vi "Constructor.vi"(6 "Database_path":path=path "D:/Sgraph_database", 8 "error in (no error)":errorcluster, 9 "DAQ-Queue":refnum<queue>, 10 "Gserver-Queue":refnum<queue>, 11 "FAMM in":refnum<class "FAMM.lvclass">) -> (0 "error out":errorcluster, 3 "FAMM out":refnum<class "FAMM.lvclass">, 5 "Layers":i32, 7 "Resolution":dbl format="%.3f")   [LabVIEW 2020, in "Sgraph_lib_V1.lvlib" / "FAMM.lvclass"]
doc: "The FAMM constructor has to be run once in order to set all historian configurations from ini files and to make all memory layer instances. Also the DBAL database type instance is created here. The FAMM object contains all references to FAMM memory and DBAL database methods."
uses:
  FAMM.lvclass
  Gserver/controls/Typedef_Gviewer-Query.ctl
  Gserver/controls/Typedef_QueryType.ctl
  HISW/controls/typedef-DAQ-datagram.ctl
  HISW/controls/typedef-Qtype.ctl
  controls/FAMM-attributes.ctl
  Common/controls/typedef_com_TagProp.ctl
  DBAL/DBAL.lvclass
  PAQ-memory.lvclass
  DBAL/controls/DBAL_Command.ctl
  DBAL/controls/DBAL-commands.ctl
  FAMM.lvclass/FAMM.ctl
  Common/controls/Global-services.vi
  Builds/Sgraph_lib_V1.lvlib
  Gserver/Gserver.lvclass
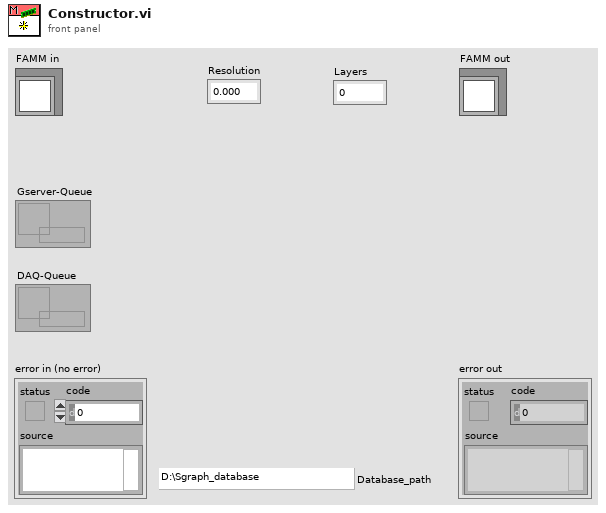
[diagram p1: front panel]
types:
  T1 = typedef "Sgraph_lib_V1.lvlib/FAMM.lvclass/FAMM-attributes.ctl" = cluster{"FAMM_PAQ_Layers":i32, "FAMM_PAQ_resolution":dbl, "PAQ_TAGs":string[], "WAQ_TAGs":string[], "EAQ_TAGs":string[], "All_TAGs":string[], "PAQtagProps":T2[], "WAQtagProps":T2[], "EAQtagProps":T2[], "DBAL_class":refnum<data-value>, "PAQ_memory":refnum<data-value>[], "PAQupdates":timestamp[], "FAMM_Size":cluster{"other":i32, "1day":i32, "1week":i32}, "DatabaseFileExtention":string, "DatabaseSaveRate":dbl, "Database_path":path, "DBAL-Queue":refnum<queue>}
  T2 = typedef "Sgraph_lib_V1.lvlib/typedef_com_TagProp.ctl" = cluster{"Description":string, "EngUnits":string, "RangeH":dbl, "RangeL":dbl, "Resolution":i32, "Obsolete":bool, "ChangeDate":timestamp, "ChangeSource":string, "ChangeReason":string, "TagFunc":u32}
  T3 = cluster{"Size":i32, "Layer":i32, "TableName":string, "LayersQTY":i32, "Skip":i32}
  T4 = typedef "Sgraph_lib_V1.lvlib/DBAL_TAGprops.ctl" = T5[]
  T5 = typedef "Sgraph_lib_V1.lvlib/DBAL_TAGpropEdit.ctl" = cluster{"TAG":string, "Qtype":string, "TAGprop":T2}
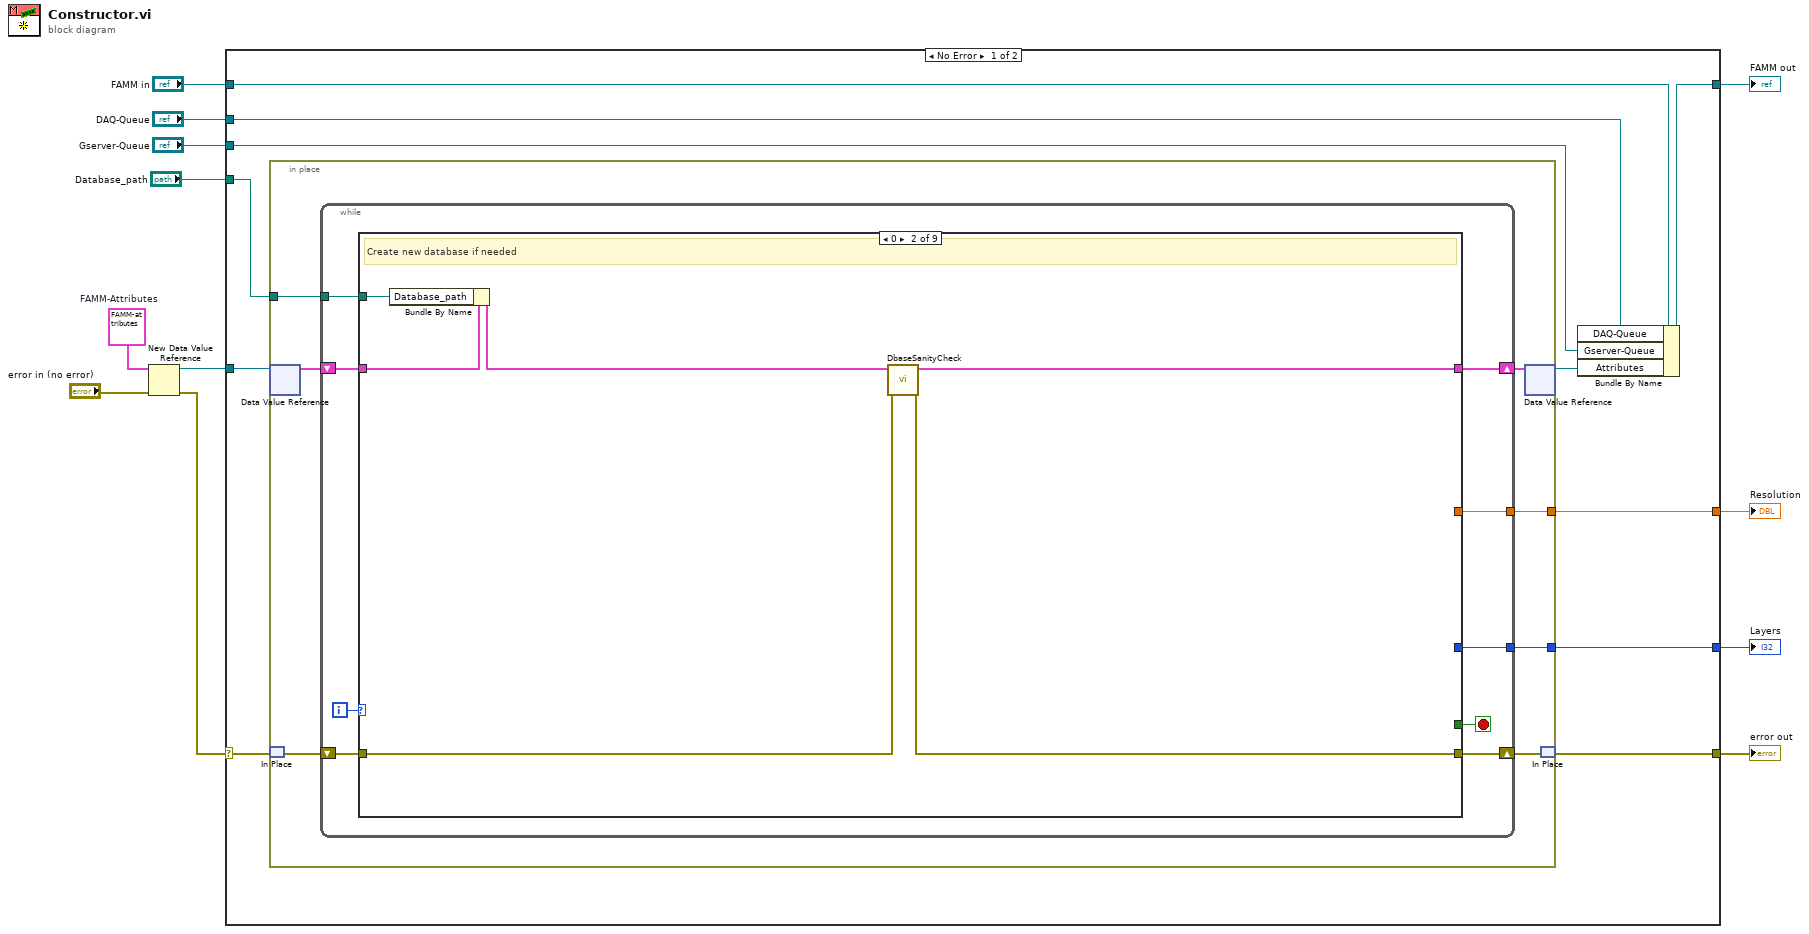
[diagram p0: block diagram]
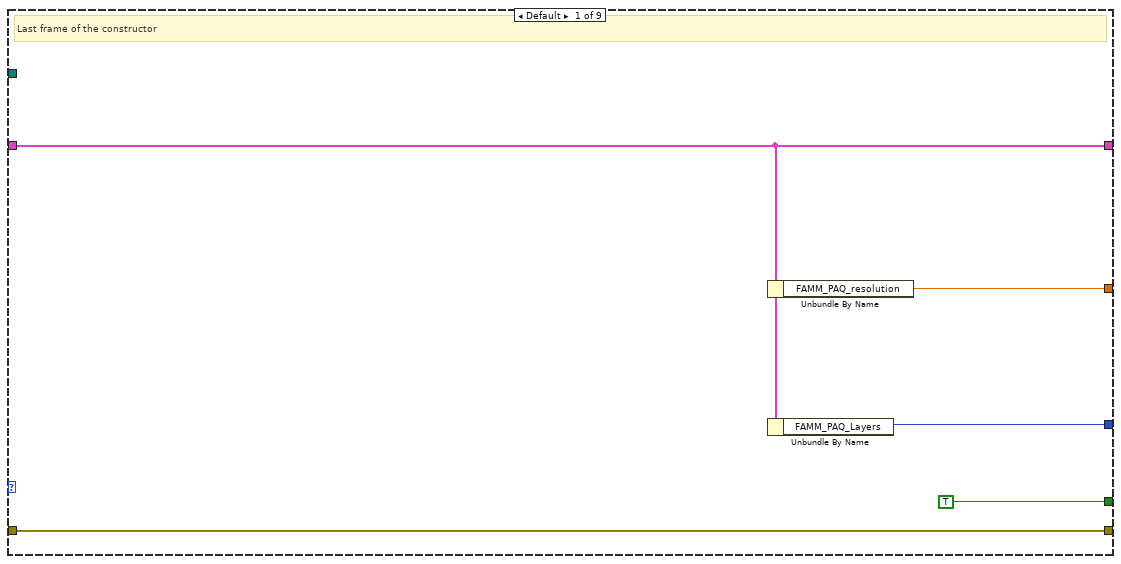
[diagram p2: hidden frame]
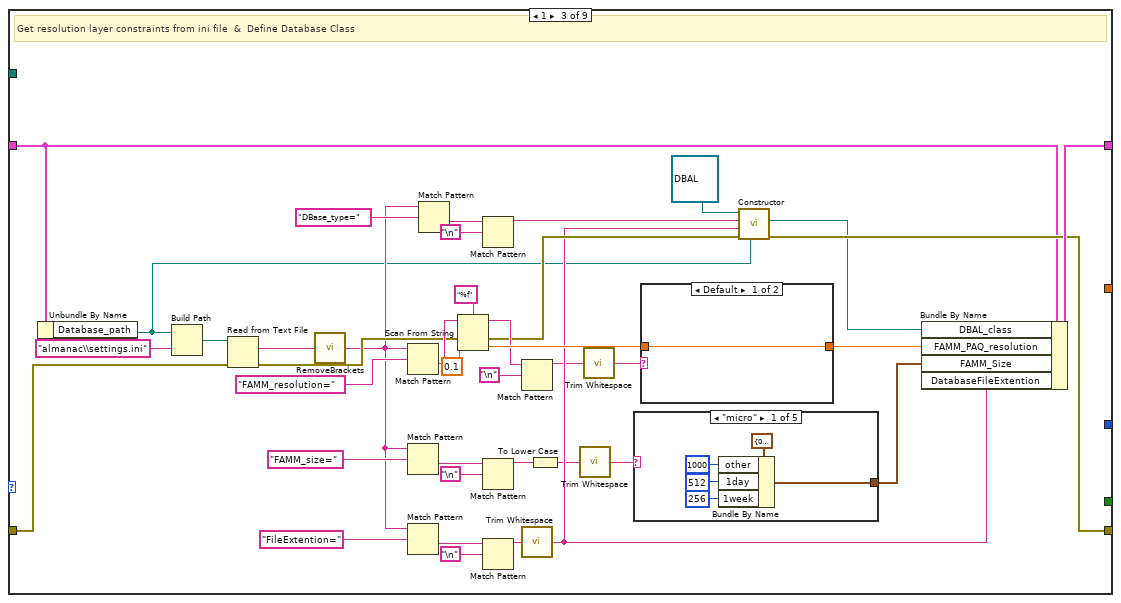
[diagram p3: hidden frame]
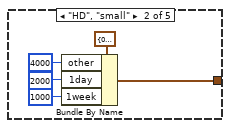
[diagram p4: hidden frame]
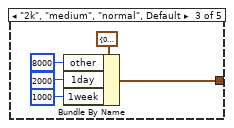
[diagram p5: hidden frame]
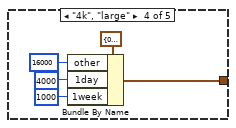
[diagram p6: hidden frame]
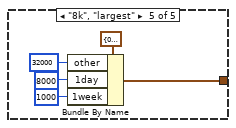
[diagram p7: hidden frame]
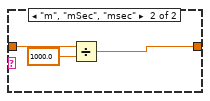
[diagram p8: hidden frame]
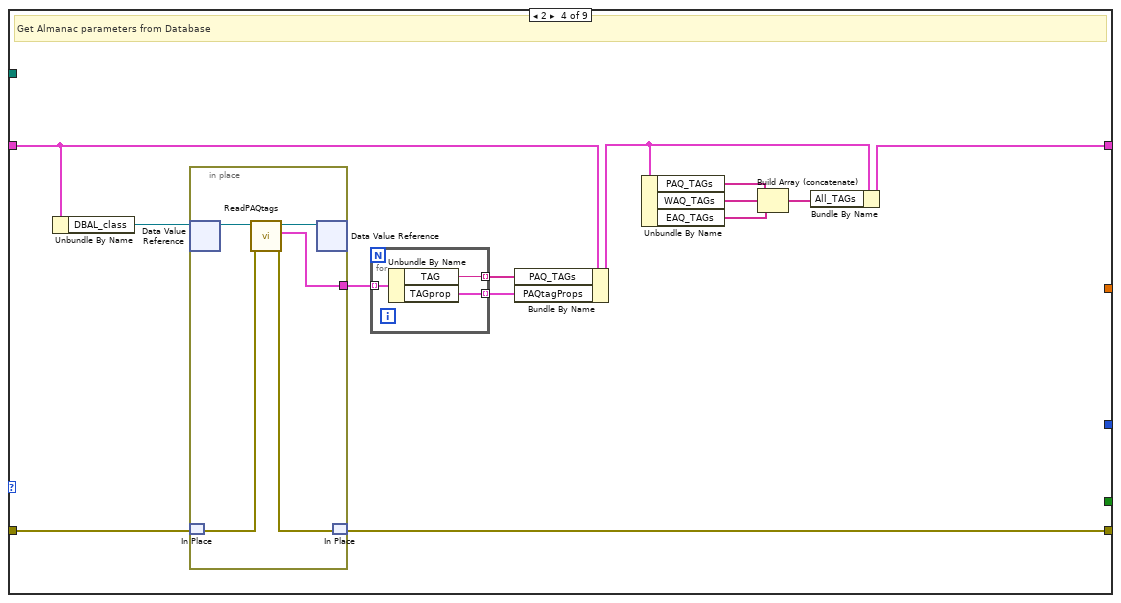
[diagram p9: hidden frame]
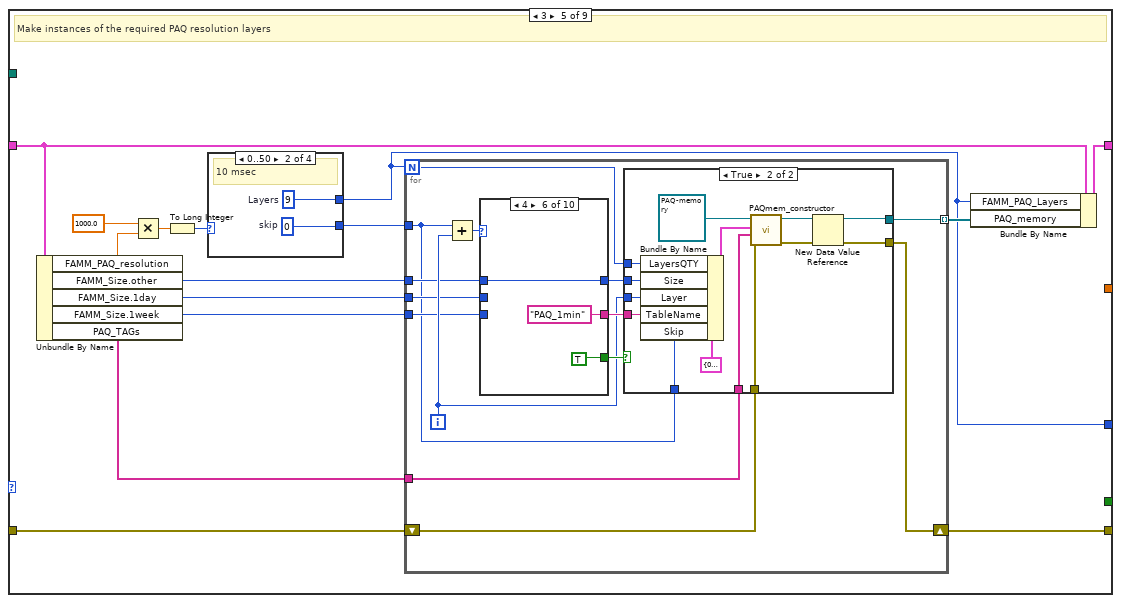
[diagram p10: hidden frame]
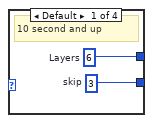
[diagram p11: hidden frame]
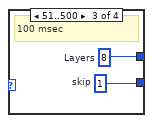
[diagram p12: hidden frame]
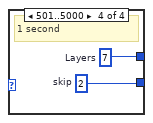
[diagram p13: hidden frame]
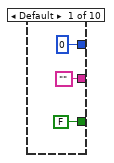
[diagram p15: hidden frame]
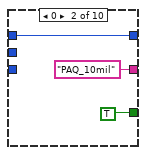
[diagram p16: hidden frame]
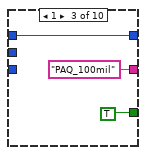
[diagram p17: hidden frame]
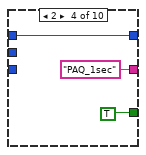
[diagram p18: hidden frame]
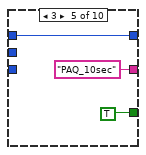
[diagram p19: hidden frame]
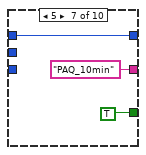
[diagram p20: hidden frame]
diagram:
  w2 = T1 {"FAMM_PAQ_Layers"=0, "FAMM_PAQ_resolution"=0.0, "PAQ_TAGs"=[], "WAQ_TAGs"=[], "EAQ_TAGs"=[], "All_TAGs"=[], "PAQtagProps"=[], "WAQtagProps"=[], "EAQtagProps"=[], "DBAL_class"=refnum, "PAQ_memory"=[], "PAQupdates"=[], "FAMM_Size"={"other"=0, "1day"=0, "1week"=0}, "DatabaseFileExtention"="", "DatabaseSaveRate"=0.0, "Database_path"=path "", "DBAL-Queue"=refnum}  # FAMM-Attributes
  n1 = New Data Value Reference(data value=w2, error in="error in (no error)") -> (data value reference=w7:refnum<data-value>, error out=w10:errorcluster)
  n2 = case shown="No Error" w10 {
    selector: w10 -> [w22 w259]
    tunnel: [w21 w259] -> w12
    tunnel: "FAMM in" -> [w14 w258]
    tunnel: [w18 w258] -> w9
    tunnel: w7 -> [w23 _]
    tunnel: [w15 _] -> w8
    tunnel: "Gserver-Queue" -> [w19 _]
    tunnel: "DAQ-Queue" -> [w17 _]
    tunnel: [w16 _] -> w3
    tunnel: "Database_path" -> [w13 _]
    frame No Error {
      n3 = in-place {
        in-place-border: [w26] -> w15
        in-place-border: [w25] -> w16
        in-place-border: w13 -> [w24]
        n4 = in-place-dvr #1(w23) -> (w30:T1)  [unwired: 1 out]
        n5 = in-place-match #2(w22) -> (w29:errorcluster)
        n6 = while {
          shift-right: [w37] -> w28
          shift-left: w30 -> [w38]
          shift-right: [w35] -> w27
          shift-left: w29 -> [w36]
          tunnel: [w33] -> w26
          tunnel: [w32] -> w25
          tunnel: w24 -> [w31]
          i -> [w39]
          stop <- w34 stop-if-true
          n7 = case shown="0" w39 {
            tunnel: w38 -> [w42 w50 w52 w120 w147 w224 w233 w235 w256]
            tunnel: [w42 w47 w80 w122 w146 w222 w232 w235 w254] -> w37
            tunnel: w36 -> [w44 w45 w70 w128 w149 w221 w231 w237 w257]
            tunnel: [w44 w46 w72 w121 w148 w221 w230 w234 w257] -> w35
            tunnel: [TRUE _ _ _ _ _ _ _ _] -> w34
            tunnel: [w40 _ _ _ _ _ _ _ _] -> w33
            tunnel: [w41 _ _ _ w140 _ _ _ _] -> w32
            tunnel: w31 -> [_ w49 _ _ _ _ _ _ _]
            frame Default {
              # "Last frame of the constructor"
              n8 = Unbundle By Name(w42) -> ("FAMM_PAQ_resolution"=w40:dbl)
              n9 = Unbundle By Name(w42) -> ("FAMM_PAQ_Layers"=w41:i32)
            }
            frame 0 {
              # "Create new database if needed"
              n10 = Bundle By Name(cluster=w50, "Database_path"=w49) -> (w48:T1)
              n11 = call "DbaseSanityCheck.vi"("error in (no error)"=w45, "FAMM in"=w48) -> ("error out"=w46:errorcluster, "FAMM out"=w47:T1)  [unwired: 8 in]
            }
            frame 1 {
              # "Get resolution layer constraints from ini file  &  Define Database Class"
              n12 = Unbundle By Name(w52) -> ("Database_path"=w51:path)
              n13 = Build Path(base path=w51, name or relative path="almanac\\settings.ini") -> (appended path=w88:path)
              n14 = Read from Text File(file (use dialog)=w88, error in=w70) -> (text=w58:string, error out=w79:errorcluster)  [unwired: 2 in, 2 out]
              n15 = call "RemoveBrackets.vi"("String in"=w58) -> ("String out"=w57:string)  [unwired: 6 in]
              n16 = Match Pattern(string=w57, regular expression="FAMM_resolution=" ("format string")) -> (after substring=w85:string)  [unwired: 1 in, 3 out]
              n17 = Match Pattern(string=w57, regular expression="FAMM_size=" ("format string")) -> (after substring=w66:string)  [unwired: 1 in, 3 out]
              n18 = Match Pattern(string=w57, regular expression="FileExtention=" ("format string")) -> (after substring=w63:string)  [unwired: 1 in, 3 out]
              n19 = Match Pattern(string=w57, regular expression="DBase_type=" ("format string")) -> (after substring=w74:string)  [unwired: 1 in, 3 out]
              n20 = Scan From String(format string="%f", input string=w85, error in=w79, default 1=0.1 ("default value 1")) -> (remaining string=w82:string, error out=w69:errorcluster, output 1=w83:dbl)  [unwired: 1 in, 1 out]
              n21 = Match Pattern(string=w74, regular expression="\n") -> (before substring=w73:string)  [unwired: 1 in, 3 out]
              n22 = Match Pattern(string=w66, regular expression="\n") -> (before substring=w65:string)  [unwired: 1 in, 3 out]
              n23 = Match Pattern(string=w63, regular expression="\n") -> (before substring=w60:string)  [unwired: 1 in, 3 out]
              n24 = Match Pattern(string=w82, regular expression="\n") -> (before substring=w56:string)  [unwired: 1 in, 3 out]
              n25 = call <vilib>:"Trim Whitespace.vi"("string"=w60) -> ("trimmed string"=w59:string)  [unwired: 1 in]
              n26 = To Lower Case(string=w65) -> (all lower case string=w54:string)
              n27 = call <vilib>:"Trim Whitespace.vi"("string"=w54) -> ("trimmed string"=w53:string)  [unwired: 1 in]
              n28 = call <vilib>:"Trim Whitespace.vi"("string"=w56) -> ("trimmed string"=w55:string)  [unwired: 1 in]
              n29 = case shown="\"micro\"" w53 {
                tunnel: [w90 w95 w100 w105 w110] -> w64
                frame "micro" {
                  n30 = Bundle By Name(cluster=cluster{"other":i32, "1day":i32, "1week":i32} {"other"=0, "1day"=0, "1week"=0} ("FAMM_Size"), "other"=1000, "1day"=512 ("other"), "1week"=256 ("other")) -> (w90:cluster{"other":i32, "1day":i32, "1week":i32})
                }
                frame "HD", "small" {
                  n31 = Bundle By Name(cluster=cluster{"other":i32, "1day":i32, "1week":i32} {"other"=0, "1day"=0, "1week"=0} ("FAMM_Size"), "other"=4000, "1day"=2000 ("other"), "1week"=1000 ("other")) -> (w95:cluster{"other":i32, "1day":i32, "1week":i32})
                }
                frame "2k", "medium", "normal", Default {
                  n32 = Bundle By Name(cluster=cluster{"other":i32, "1day":i32, "1week":i32} {"other"=0, "1day"=0, "1week"=0} ("FAMM_Size"), "other"=8000, "1day"=2000 ("other"), "1week"=1000 ("other")) -> (w100:cluster{"other":i32, "1day":i32, "1week":i32})
                }
                frame "4k", "large" {
                  n33 = Bundle By Name(cluster=cluster{"other":i32, "1day":i32, "1week":i32} {"other"=0, "1day"=0, "1week"=0} ("FAMM_Size"), "other"=16000, "1day"=4000 ("other"), "1week"=1000 ("other")) -> (w105:cluster{"other":i32, "1day":i32, "1week":i32})
                }
                frame "8k", "largest" {
                  n34 = Bundle By Name(cluster=cluster{"other":i32, "1day":i32, "1week":i32} {"other"=0, "1day"=0, "1week"=0} ("FAMM_Size"), "other"=32000, "1day"=8000 ("other"), "1week"=1000 ("other")) -> (w110:cluster{"other":i32, "1day":i32, "1week":i32})
                }
              }
              n35 = case shown="Default" w55 {
                tunnel: w83 -> [w115 w118]
                tunnel: [w115 w116] -> w81
                frame Default {
                }
                frame "m", "mSec", "msec" {
                  n36 = Divide(x=w118, y=1000.0) -> (x/y=w116:dbl)
                }
              }
              n37 = call "Constructor.vi"("Database_location"=w51, "error in (no error)"=w69, "File extention"=w59, "DatabaseType"=w73, "DBAL in"=refnum<class "DBAL.lvclass"> refnum) -> ("error out"=w72:errorcluster, "DBAL_class"=w71:refnum<data-value>)  [unwired: 4 in, 1 out]
              n38 = Bundle By Name(cluster=w52, "DBAL_class"=w71, "FAMM_PAQ_resolution"=w81, "FAMM_Size"=w64, "DatabaseFileExtention"=w59) -> (w80:T1)
            }
            frame 2 {
              # "Get Almanac parameters from Database"
              n39 = Unbundle By Name(w120) -> ("DBAL_class"=w119:refnum<data-value>)
              n40 = in-place {
                in-place-border: [w135] -> w131
                n41 = in-place-dvr #3(w119) -> (w139:refnum<class "DBAL.lvclass">)  [unwired: 1 out]
                n42 = in-place-match #4(w128) -> (w138:errorcluster)
                n43 = call-dynamic "ReadPAQtags.vi"("error in (no error)"=w138, "DBAL in"=w139) -> ("error out"=w137:errorcluster, "PAQ_TAGs"=w135:T4, "DBAL out"=w136:refnum<class "DBAL.lvclass">)  [unwired: 7 in]
                n44 = in-place-dvr #3(w136) -> ()  [unwired: 2 out]
                n45 = in-place-match #4(w137) -> (w121:errorcluster)
              }
              n46 = for {
                tunnel: w131 -> [w134] mode=indexing
                tunnel: [w133] -> w130 mode=indexing
                tunnel: [w132] -> w129 mode=indexing
                n47 = Unbundle By Name(w134) -> ("TAG"=w133:string, "TAGprop"=w132:T2)
              }
              n48 = Bundle By Name(cluster=w120, "PAQ_TAGs"=w130, "PAQtagProps"=w129) -> (w123:T1)
              n49 = Unbundle By Name(w123) -> ("PAQ_TAGs"=w127:string[], "WAQ_TAGs"=w126:string[], "EAQ_TAGs"=w125:string[])
              n50 = Build Array (concatenate)(w127, w126, w125) -> (w124:string[])
              n51 = Bundle By Name(cluster=w123, "All_TAGs"=w124) -> (w122:T1)
            }
            frame 3 {
              # "Make instances of the required PAQ resolution layers"
              n52 = Unbundle By Name(w147) -> ("FAMM_PAQ_resolution"=w154:dbl, "FAMM_Size.other"=w143:i32, "FAMM_Size.1day"=w141:i32, "FAMM_Size.1week"=w142:i32, "PAQ_TAGs"=w144:string[])
              n53 = Multiply(x=1000.0, y=w154) -> (x*y=w152:dbl)
              n54 = To Long Integer(number=w152) -> (32bit integer=w151:i32)
              n55 = case shown="0..50" w151 {
                tunnel: [w156 w158 w160 w162] -> w150
                tunnel: [w155 w157 w159 w161] -> w140
                frame Default {
                  w155 = 6  # Layers
                  w156 = 3  # skip
                  # "10 second and up"
                }
                frame 0..50 {
                  w157 = 9  # Layers
                  w158 = 0  # skip
                  # "10 msec"
                }
                frame 51..500 {
                  w159 = 8  # Layers
                  w160 = 1  # skip
                  # "100 msec"
                }
                frame 501..5000 {
                  w161 = 7  # Layers
                  w162 = 2  # skip
                  # "1 second"
                }
              }
              n56 = for {
                N: w140 -> [w166]
                tunnel: w150 -> [w163]
                shift-right: [w170] -> w148
                shift-left: w149 -> [w176]
                tunnel: [w169] -> w145 mode=indexing
                tunnel: w143 -> [w168]
                tunnel: w144 -> [w167]
                tunnel: w142 -> [w165]
                tunnel: w141 -> [w164]
                i -> [w171]
                n57 = Add(x=w163, y=w171) -> (x+y=w175:i32)
                n58 = case shown="4" w175 {
                  tunnel: [0 ("Size") w194 w197 w200 w203 w206 w209 w212 w215 w218] -> w174
                  tunnel: [FALSE TRUE TRUE TRUE TRUE TRUE TRUE TRUE TRUE TRUE] -> w173
                  tunnel: ["" "PAQ_10mil" "PAQ_100mil" "PAQ_1sec" "PAQ_10sec" "PAQ_1min" "PAQ_10min" "PAQ_2hr" "PAQ_1day" "PAQ_1wk"] -> w172
                  tunnel: w168 -> [_ w194 w197 w200 w203 w206 w209 w212 _ _]
                  tunnel: w165 -> [_ _ _ _ _ _ _ _ _ w218]
                  tunnel: w164 -> [_ _ _ _ _ _ _ _ w215 _]
                  frame Default {
                  }
                  frame 0 {
                  }
                  frame 1 {
                  }
                  frame 2 {
                  }
                  frame 3 {
                  }
                  frame 4 {
                  }
                  frame 5 {
                  }
                  frame 6 {
                  }
                  frame 7 {
                  }
                  frame 8 {
                  }
                }
                n59 = case shown="True" w173 {
                  tunnel: w176 -> [_ w189]
                  tunnel: w174 -> [_ w188]
                  tunnel: w171 -> [_ w187]
                  tunnel: w172 -> [_ w186]
                  tunnel: [_ w182] -> w170
                  tunnel: [_ w183] -> w169
                  tunnel: w167 -> [_ w181]
                  tunnel: w166 -> [_ w178]
                  tunnel: w163 -> [_ w177]
                  frame False {
                  }
                  frame True {
                    n60 = Bundle By Name(cluster=T3 {"Size"=0, "Layer"=0, "TableName"="", "LayersQTY"=0, "Skip"=0} ("LayerInfo"), "LayersQTY"=w178, "Size"=w188, "Layer"=w187, "TableName"=w186, "Skip"=w177) -> (w179:T3)
                    n61 = call-dynamic "PAQmem_constructor.vi"("error in (no error)"=w189, "TAGs"=w181, "LayerInfo"=w179, "PAQ-memory in"=refnum<class "PAQ-memory.lvclass"> refnum) -> ("error out"=w184:errorcluster, "PAQ-memory out"=w185:refnum<class "PAQ-memory.lvclass">)  [unwired: 6 in]
                    n62 = New Data Value Reference(data value=w185, error in=w184) -> (data value reference=w183:refnum<data-value>, error out=w182:errorcluster)
                  }
                }
              }
              n63 = Bundle By Name(cluster=w147, "FAMM_PAQ_Layers"=w140, "PAQ_memory"=w145) -> (w146:T1)
            }
            frame 4 {
              # "Determine the speed to periodically update database content"
              n64 = Unbundle By Name(w224) -> ("FAMM_PAQ_resolution"=w226:dbl)
              n65 = Multiply(x=w226, y=100.0) -> (x*y=w227:dbl)
              n66 = In Range and Coerce "Database\nsave pace"(upper limit=60.0, x=w227, lower limit=5.0) -> (coerced(x)=w223:dbl)  [unwired: 1 out]
              n67 = Bundle By Name(cluster=w224, "DatabaseSaveRate"=w223) -> (w222:T1)
            }
            frame 5 {
              # "Load existing database PAQ content into memory"
              n68 = call "PAQ_Retrieve_latest_DB_data.vi"("error in (no error)"=w231, "FAMM-Attributes in"=w233) -> ("error out"=w230:errorcluster, "FAMM-Attributes out"=w232:T1)  [unwired: 8 in]
            }
            frame 6 {
              # "Start DBAL service (for DBAL database write buffer)"
              n69 = Unbundle By Name(w235) -> ("DBAL_class"=w236:refnum<data-value>)
              n70 = in-place {
                n71 = in-place-dvr #5(w236) -> (w253:refnum<class "DBAL.lvclass">)  [unwired: 1 out]
                n72 = in-place-match #6(w237) -> (w252:errorcluster)
                n73 = call "DBAL-GetVIpath.vi"("error in (no error)"=w252, "DBAL in"=w253) -> ("error out"=w245:errorcluster, "MethodsPath"=w250:path, "DBAL out"=w246:refnum<class "DBAL.lvclass">)  [unwired: 7 in]
                n74 = Build Path(base path=w250, name or relative path="DBAL-Service.vi") -> (appended path=w249:path)
                n75 = Open VI Reference(vi path=w249, error in (no error)=w245) -> (vi reference=w248:refnum<vi>, error out=w244:errorcluster)  [unwired: 4 in]
                n76 = invoke class="VI" method="Ctrl Val.Set"(reference=w248, error in=w244, "Control Name"="DBAL_in", "Value"=w246) -> (reference out=w241:refnum<vi>, error out=w240:errorcluster)  [unwired: 1 in, 3 out]
                n77 = invoke class="VI" method="Run VI"(reference=w241, error in=w240, "Wait until done"=FALSE ("Wait Until Done"), "Auto Dispose Ref"=TRUE ("Auto Dispose Reference")) -> (reference out=w238:refnum<vi>, error out=w239:errorcluster)  [unwired: 1 in, 3 out]
                n78 = global write "Global-services.vi" "DBAL-service"(w238) -> ()
                n79 = in-place-dvr #5(w246) -> ()  [unwired: 2 out]
                n80 = in-place-match #6(w239) -> (w234:errorcluster)
              }
            }
            frame 7 {
              # "Obtain DBAL Queue"
              n81 = call "Obtain-DBAL-Queue.vi"() -> ("DBAL-Queue"=w255:refnum<queue>)  [unwired: 7 in]
              n82 = Bundle By Name(cluster=w256, "DBAL-Queue"=w255) -> (w254:T1)
            }
          }
        }
        n83 = in-place-dvr #1(w28) -> (w20:refnum<data-value>)  [unwired: 1 out]
        n84 = in-place-match #2(w27) -> (w21:errorcluster)
      }
      n85 = Bundle By Name(cluster=w14, "DAQ-Queue"=w17, "Gserver-Queue"=w19, "Attributes"=w20) -> (w18:refnum<class "FAMM.lvclass">)
    }
    frame Error {
    }
  }
  "error out" <- w12
  "FAMM out" <- w9
  "Resolution" <- w8
  "Layers" <- w3
